vi "CSE ISP - Load text file.vi"(6 "pattern":string, 7 "prompt":string, 8 "error in":errorcluster, 9 "default name":string, 11 "path":path) -> (0 "error out":errorcluster, 1 "cancelled":bool, 2 "data":string, 3 "path out":path)   [LabVIEW 2021]
doc: "::: CalcExpress Toolkit :::\nCopyright (c) 2000-2026 Konstantin Shifershteyn. All rights reserved."
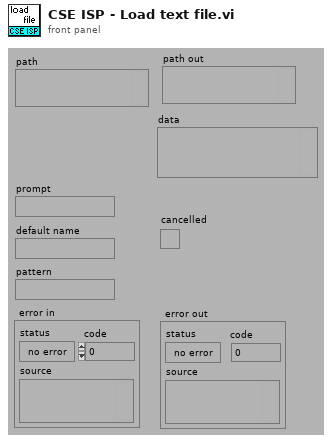
[diagram p1: front panel]
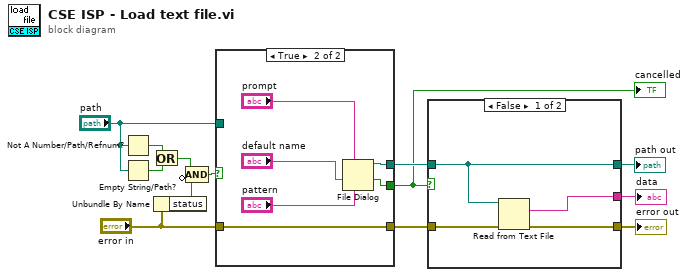
[diagram p0: block diagram]
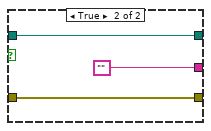
[diagram p2: hidden frame]
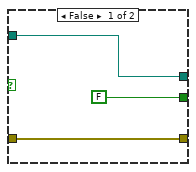
[diagram p3: hidden frame]
diagram:
  n1 = Not A Number/Path/Refnum?(number/path/refnum="path") -> (NaN/Path/Refnum?=w7:bool)
  n2 = Empty String/Path?(string/path="path") -> (empty?=w6:bool)
  n3 = Or(x=w7, y=w6) -> (x .or. y?=w5:bool)
  n4 = Unbundle By Name("error in") -> ("status"=w10:bool)
  n5 = Compound Arithmetic op=AND(w5, invert w10) -> (w8:bool)
  n6 = case shown="True" w8 {
    tunnel: [w15 w19] -> w4
    tunnel: [w16 w18] -> w12
    tunnel: "error in" -> [w16 w18]
    tunnel: "path" -> [w15 _]
    tunnel: [FALSE ("cancelled") w17] -> w1
    frame False {
    }
    frame True {
      n7 = File Dialog(6:"pattern", 7:"prompt", 9:"default name") -> (1:w17:bool, 3:w19:path)  [unwired: 4 in, 2 out]
    }
  }
  "cancelled" <- w1
  n8 = case shown="False" w1 {
    tunnel: [w25 w28] -> w2
    tunnel: [w24 ""] -> w13
    tunnel: w12 -> [w26 w28]
    tunnel: w4 -> [w23 w29]
    tunnel: [w23 w29] -> w3
    frame False {
      n9 = Read from Text File(file (use dialog)=w23, error in=w26) -> (text=w24:string, error out=w25:errorcluster)  [unwired: 2 in, 2 out]
    }
    frame True {
    }
  }
  "error out" <- w2
  "data" <- w13
  "path out" <- w3
